vi "ASD Signal Analysis VI.vi"(11 "S txt":dbl[](array[numeric])) -> (0 "Omit STD (pA)":dbl format="%0.6f", 1 "BL (pA)":dbl, 3 "S Analysis":T1)   [LabVIEW 2018]
uses:
  <vilib>/Analysis/baseanly.llb/Multimode.vi
  <vilib>/Analysis/NI_AALBase.lvlib
  <vilib>/Analysis/NI_AAL_SigProc.lvlib
panel:
  out "STD (pA)":dbl format="%0.6f"
  out "width 2":i32=5
  out "threshold 2":dbl=5.0 format="%#_13g"
  in  "threshold":dbl=5.0 format="%#_13g"
  out "width":i32=5
  out "intervals 2":i32=10
  out "intervals":i32=50
  out "サイズ":i32
  out "H2":i32 caption="検出数"
  out "H1":i32 caption="検出数"
  out "Histogram Graph 2":T2(graph) caption="ヒストグラムグラフ"
  out "Histogram Graph":T2(graph) caption="ヒストグラムグラフ"
  out "Signal R":cluster{i32[], "部分配列":dbl[]}(graph)
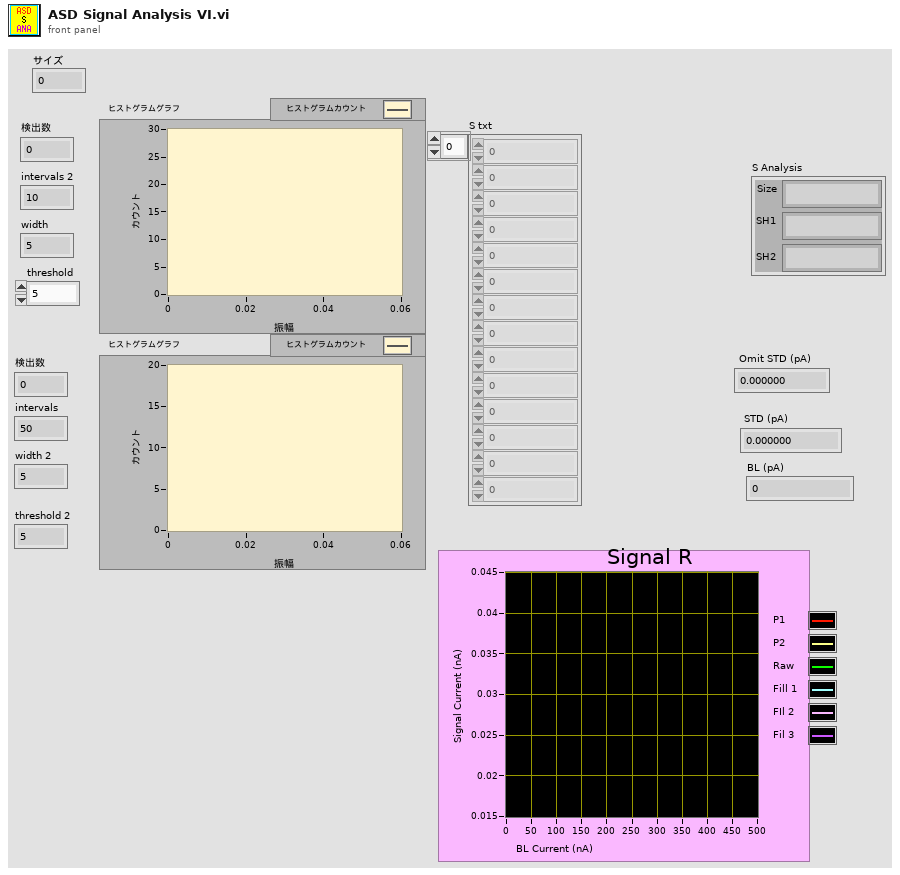
[diagram p1: front panel]
types:
  T1 = cluster{"Size":string, "SH1":string, "SH2":string}
  T2 = cluster{"X Values":dbl[], "Histogram: h(x)":i32[]}
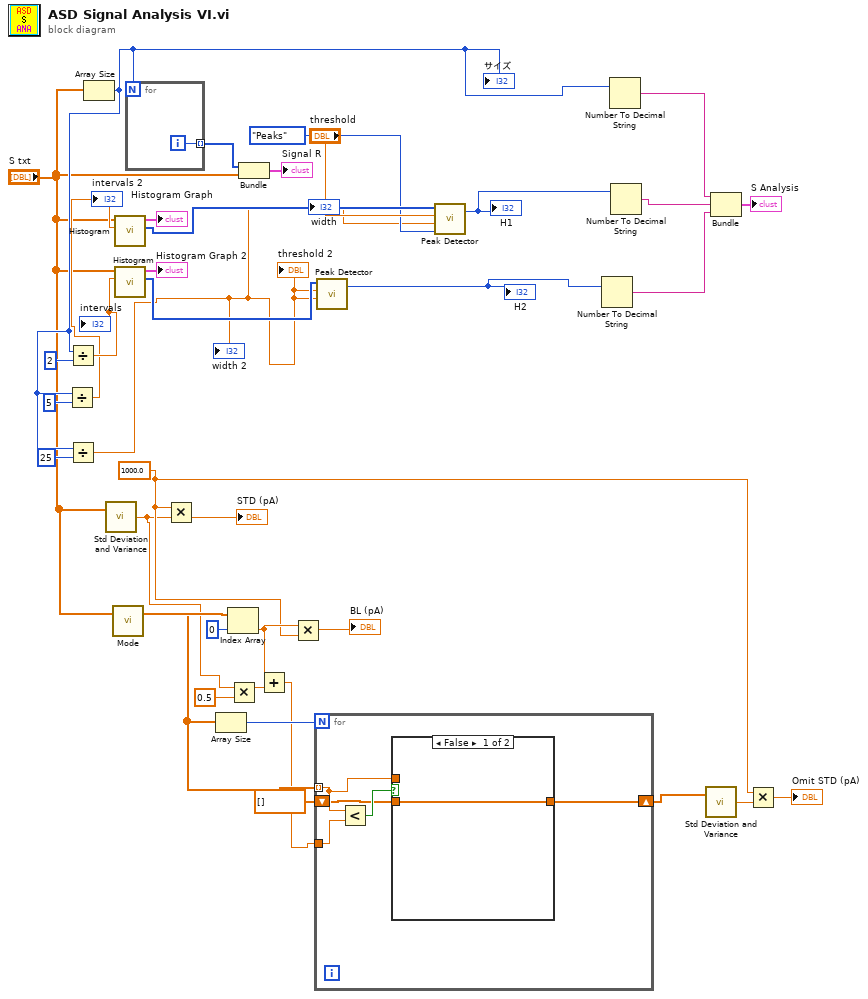
[diagram p0: block diagram]
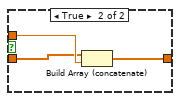
[diagram p2: hidden frame]
diagram:
  w4 = 1000.0 ("x")
  n1 = Array Size(array="S txt") -> (size(s)=w23:i32)
  "サイズ" <- w23
  n2 = Divide(x=w23, y=5) -> (x/y=w27:dbl)
  "intervals 2" <- w27
  n3 = Divide(x=w23, y=2) -> (x/y=w29:dbl)
  "intervals" <- w29
  n4 = Divide(x=w23, y=25) -> (x/y=w24:dbl)
  "width" <- w24
  "threshold 2" <- w24
  "width 2" <- w24
  n5 = call <vilib>:"Std Deviation and Variance.vi"("X"="S txt") -> ("standard deviation"=w1:dbl)  [unwired: 1 in, 2 out]
  n6 = call-poly <vilib>:"Mode.vi"("X"="S txt") -> ("Modes"=w16:dbl[])  [unwired: 1 in, 1 out]
  n7 = call <vilib>:"Histogram.vi"("intervals"=w27, "X"="S txt") -> ("Histogram: h(x)"=w33:i32[], "Histogram Graph"=→"Histogram Graph":T2)  [unwired: 6 in, 2 out]
  n8 = call <vilib>:"Histogram.vi"("intervals"=w29, "X"="S txt") -> ("Histogram: h(x)"=w25:i32[], "Histogram Graph"=→"Histogram Graph 2":T2)  [unwired: 6 in, 2 out]
  n9 = for {
    N: w23 -> [_]
    tunnel: [w38] -> w37 mode=indexing
    i -> [w38]
  }
  n10 = Multiply(x=w4, y=w1) -> (x*y=→"STD (pA)":dbl)
  n11 = Array Size(array="S txt") -> (size(s)=w13:i32)
  n12 = Index Array(array=w16, index=0 ("指標")) -> (element=w11:dbl)
  n13 = Multiply(x=w1, y=0.5) -> (x*y=w3:dbl)
  n14 = Bundle(w37, "S txt"="S txt") -> (→"Signal R":cluster{i32[], "S txt":dbl[]})  [unwired: 1 in]
  n15 = Add(x=w11, y=w3) -> (x+y=w9:dbl)
  n16 = Multiply(x=w11, y=w4) -> (x*y=→"BL (pA)":dbl)
  n17 = for {
    N: w13 -> [_]
    tunnel: "S txt" -> [w41] mode=indexing
    tunnel: w9 -> [w43]
    shift-right: [w40] -> w7
    shift-left: dbl[] [] -> [w39]
    n18 = Less?(x=w41, y=w43) -> (x < y?=w42:bool)
    n19 = case shown="False" w42 {
      tunnel: w41 -> [_ w47]
      tunnel: [w44 w46] -> w40
      tunnel: w39 -> [w44 w45]
      frame False {
      }
      frame True {
        n20 = Build Array (concatenate)(w45, w47) -> (w46:dbl[])
      }
    }
  }
  n21 = call <vilib>:"Peak Detector.vi"("width"=w24, "threshold"=w24, "X"=w25) -> ("# found"=w21:i32)  [unwired: 4 in, 4 out]
  "H2" <- w21
  n22 = call <vilib>:"Peak Detector.vi"("peaks/valleys"=enum32{"Peaks", "Valleys"}."Peaks", "width"=w24, "threshold"="threshold", "X"=w33) -> ("# found"=w22:i32)  [unwired: 3 in, 4 out]
  "H1" <- w22
  n23 = Number To Decimal String(number=w21) -> (decimal integer string=w18:string)  [unwired: 1 in]
  n24 = Number To Decimal String(number=w23) -> (decimal integer string=w20:string)  [unwired: 1 in]
  n25 = Number To Decimal String(number=w22) -> (decimal integer string=w19:string)  [unwired: 1 in]
  n26 = call <vilib>:"Std Deviation and Variance.vi"("X"=w7) -> ("standard deviation"=w6:dbl)  [unwired: 1 in, 2 out]
  n27 = Bundle(w20, w19, w18) -> (→"S Analysis":cluster{string, string, string})  [unwired: 1 in]
  n28 = Multiply(x=w4, y=w6) -> (x*y=→"Omit STD (pA)":dbl)
